vi "Connect RF Switch Box.vi"(8 "error in (no error)":errorcluster caption="에러 입력(에러 없음)", 9 "포트":u16, 10 "주소":string, 11 "Instrument Manager 입력":refnum<class "Instrument Manager.lvclass">) -> (0 "error out":errorcluster caption="에러 출력", 3 "Instrument Manager 출력":refnum<class "Instrument Manager.lvclass">)   [LabVIEW 2023, in "Instrument Manager.lvclass"]
uses:
  Instrument Manager.lvclass
  Instrument Manager.lvclass/Instrument Manager.ctl
  Module/CE RF Switch Box/CE RF Switch Box/CE RF Switch Box.lvclass
  C:/Users/HCT-3320/Documents/Instrument Manger/Module/CE RF Switch Box/CE RF Switch Box/CE RF Switch Box.lvclass
  C:/Users/HCT-3320/Documents/Instrument Manger/Module/CE RF Switch Box/RF Filter Box/RF Filter Box.lvclass
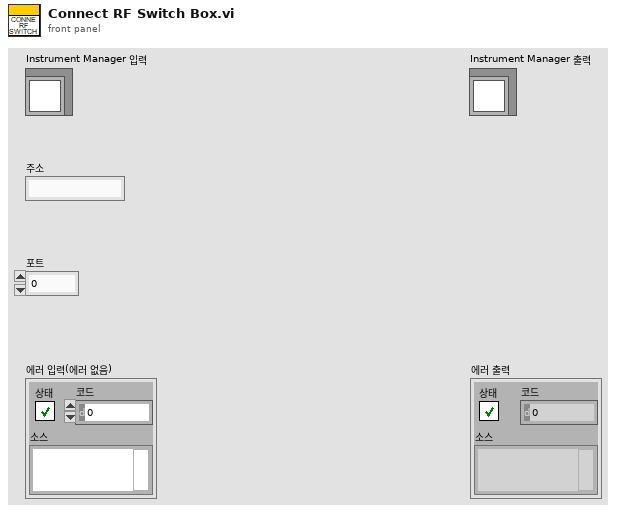
[diagram p1: front panel]
types:
  T1 = cluster{"Anritsu Call Box":refnum<class "Anritsu Call Box.lvclass">, "Spectrum Analyzer":refnum<class "Interface_Spectrum.lvclass">, "RF Switch Box":refnum<class "RF Filter Box.lvclass">, "Turn Table":refnum<class "Interface - Turn Table.lvclass">, "Mast":refnum<class "Interface - Mast.lvclass">, "3D Controller":refnum<class "Interface_3D Controller.lvclass">}
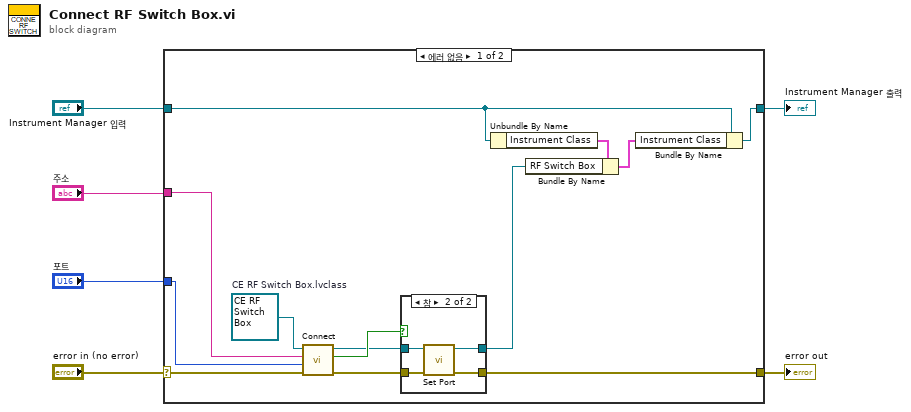
[diagram p0: block diagram]
diagram:
  n1 = case shown="에러 없음" "error in (no error)" {
    selector: "error in (no error)" -> [w14 w27]
    tunnel: [w9 w27] -> w5
    tunnel: [w19 w26] -> w3
    tunnel: "Instrument Manager 입력" -> [w18 w26]
    tunnel: "포트" -> [w8 _]
    tunnel: "주소" -> [w7 _]
    frame No Error {
      w15 = refnum<class "CE RF Switch Box.lvclass"> refnum  # CE RF Switch Box.lvclass
      n2 = call-dynamic "Connect.vi"("error in (no error)"=w14, "원격 포트 또는 서비스 이름"=w8, "주소"=w7, "CE RF Switch Box 입력"=w15) -> ("error out"=w12:errorcluster, "Connected?"=w13:bool, "CE RF Switch Box 출력"=w11:refnum<class "CE RF Switch Box.lvclass">)  [unwired: 5 in]
      n3 = case shown="참" w13 {
        tunnel: w12 -> [w20 w25]
        tunnel: w11 -> [w21 w24]
        tunnel: [w21 w23] -> w10
        tunnel: [w20 w22] -> w9
        frame False {
        }
        frame True {
          n4 = call "Set Port.vi"("error in (no error)"=w25, "CE RF Switch Box 입력"=w24) -> ("error out"=w22:errorcluster, "CE RF Switch Box 출력"=w23:refnum<class "CE RF Switch Box.lvclass">)  [unwired: 8 in]
        }
      }
      n5 = Unbundle By Name(w18) -> ("Instrument Class"=w17:T1)
      n6 = Bundle By Name(cluster=w17, "RF Switch Box"=w10) -> (w16:T1)
      n7 = Bundle By Name(cluster=w18, "Instrument Class"=w16) -> (w19:refnum<class "Instrument Manager.lvclass">)
    }
    frame Error {
    }
  }
  "error out" <- w5
  "Instrument Manager 출력" <- w3
